vi "Get Empty Row.vi"(8 "error in (no error)":errorcluster, 11 "Result Handler":refnum<class "TestStand Result Handler.lvclass">) -> (0 "error out":errorcluster, 2 "Empty Row":string[](array[string]), 3 "Result Handler":refnum<class "TestStand Result Handler.lvclass">)   [LabVIEW 2020, in "Astemes_CSVReportPlugin.lvlib" / "TestStand Result Handler.lvclass"]
uses:
  TestStand Result Handler.lvclass
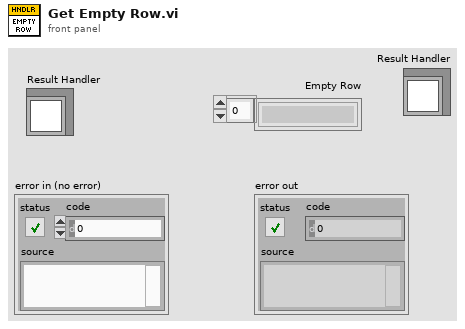
[diagram p1: front panel]
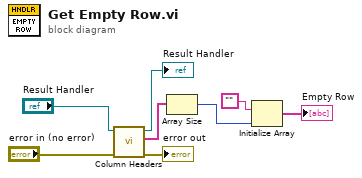
[diagram p0: block diagram]
diagram:
  n1 = call-dynamic "Column Headers.vi"("error in (no error)"="error in (no error)", "TestStand Result Handler in"="Result Handler") -> ("error out"=→"error out":errorcluster, "Array"=w3:string[], "TestStand Result Handler out"=→"Result Handler":refnum<class "TestStand Result Handler.lvclass">)  [unwired: 7 in]
  n2 = Array Size(array=w3) -> (size(s)=w7:i32)
  n3 = Initialize Array("", w7) -> (→"Empty Row":string[])
